vi "CO tune TurnTable Angle.vi"(8 "error in (no error)":errorcluster caption="에러 입력(에러 없음)", 11 "Instrument Manager 입력":refnum<class "Instrument Manager.lvclass">) -> (0 "error out":errorcluster caption="에러 출력", 3 "Instrument Manager 출력":refnum<class "Instrument Manager.lvclass">)   [LabVIEW 2023, in "Instrument Manager.lvclass"]
uses:
  Instrument Manager.lvclass
  Instrument Manager.lvclass/Instrument Manager.ctl
  Module/Turn Table and Mast Control/Interface Class/Turn Table/Interface - Turn Table.lvclass
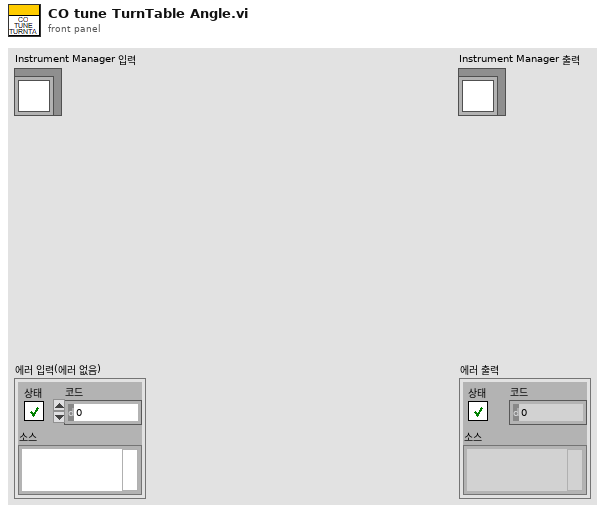
[diagram p1: front panel]
types:
  T1 = cluster{"Anritsu Call Box":refnum<class "Anritsu Call Box.lvclass">, "Spectrum Analyzer":refnum<class "Interface_Spectrum.lvclass">, "RF Switch Box":refnum<class "RF Filter Box.lvclass">, "Turn Table":refnum<class "Interface - Turn Table.lvclass">, "Mast":refnum<class "Interface - Mast.lvclass">, "3D Controller":refnum<class "Interface_3D Controller.lvclass">}
  T2 = cluster{"Target Angle":dbl, "Turn Table Speed":i32, "Fetch Interval":i32}
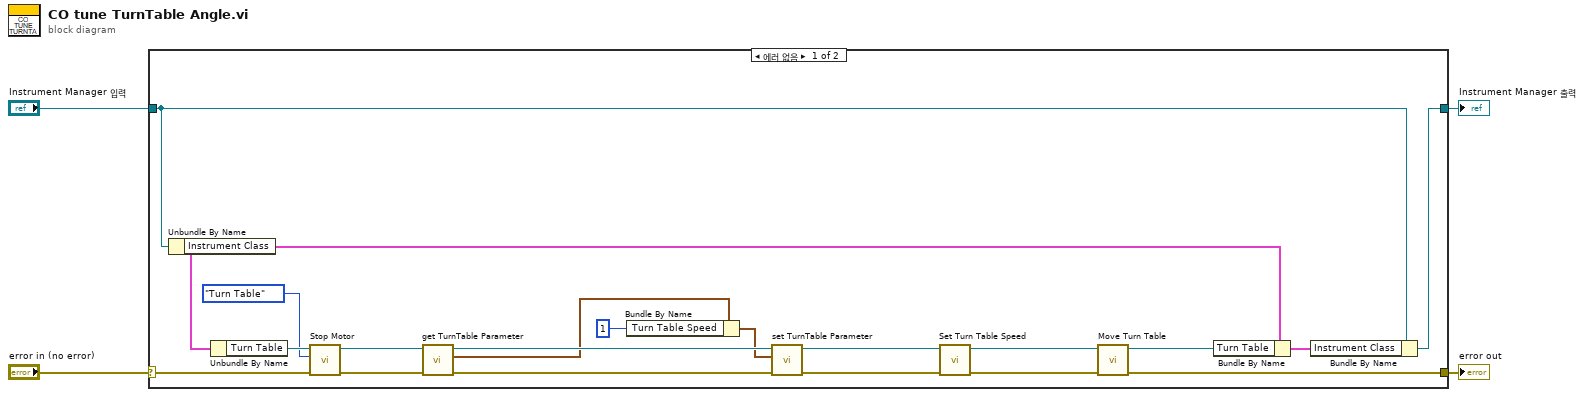
[diagram p0: block diagram]
diagram:
  n1 = case shown="에러 없음" "error in (no error)" {
    selector: "error in (no error)" -> [w14 w26]
    tunnel: [w20 w26] -> w3
    tunnel: [w5 w25] -> w1
    tunnel: "Instrument Manager 입력" -> [w7 w25]
    frame No Error {
      n2 = Unbundle By Name(w7) -> ("Instrument Class"=w9:T1)
      n3 = Unbundle By Name(w9) -> ("Turn Table"=w11:refnum<class "Interface - Turn Table.lvclass">)
      n4 = call-dynamic "Stop Motor.vi"("error in (no error)"=w14, "Target"=enum16{"Mast", "Turn Table"}."Turn Table", "Interface - Turn Table in"=w11) -> ("error out"=w13:errorcluster, "Interface - Turn Table out"=w12:refnum<class "Interface - Turn Table.lvclass">)  [unwired: 7 in]
      n5 = call-dynamic "get TurnTable Parameter.vi"("error in (no error)"=w13, "Interface - Turn Table 입력"=w12) -> ("error out"=w19:errorcluster, "Turn Table Info"=w17:T2, "Interface - Turn Table 출력"=w18:refnum<class "Interface - Turn Table.lvclass">)  [unwired: 7 in]
      n6 = Bundle By Name(cluster=w17, "Turn Table Speed"=1) -> (w15:T2)
      n7 = call-dynamic "set TurnTable Parameter.vi"("error in (no error)"=w19, "Turn Table Info"=w15, "Interface - Turn Table in"=w18) -> ("error out"=w22:errorcluster, "Interface - Turn Table out"=w24:refnum<class "Interface - Turn Table.lvclass">)  [unwired: 7 in]
      n8 = call-dynamic "Set Turn Table Speed.vi"("error in (no error)"=w22, "Interface - Turn Table in"=w24) -> ("error out"=w21:errorcluster, "Interface - Turn Table out"=w23:refnum<class "Interface - Turn Table.lvclass">)  [unwired: 8 in]
      n9 = call-dynamic "Move Turn Table.vi"("error in (no error)"=w21, "Interface - Turn Table in"=w23) -> ("error out"=w20:errorcluster, "Interface - Turn Table out"=w8:refnum<class "Interface - Turn Table.lvclass">)  [unwired: 8 in]
      n10 = Bundle By Name(cluster=w9, "Turn Table"=w8) -> (w6:T1)
      n11 = Bundle By Name(cluster=w7, "Instrument Class"=w6) -> (w5:refnum<class "Instrument Manager.lvclass">)
    }
    frame Error {
    }
  }
  "error out" <- w3
  "Instrument Manager 출력" <- w1
